vi "Write Outputs.vi"(8 "error in (no error)":errorcluster, 10 "Analog Outputs":sgl[](array[numeric]), 11 "An Out in":refnum<class "M5StackDAC2.lvclass">) -> (0 "error out":errorcluster, 3 "An Out out":refnum<class "M5StackDAC2.lvclass">)   [LabVIEW 2020, in "CTI-Peripheral.lvlib" / "M5StackDAC2.lvclass"]
uses:
  M5StackDAC2.lvclass
  M5StackDAC2.lvclass/M5StackDAC2.ctl
  CTI/I2C Connection/I2C Connection.lvclass/I2C Connection.ctl
  CTI/Session/I2C Write Data.vi
  CTI/I2C Connection/I2C Connection.lvclass
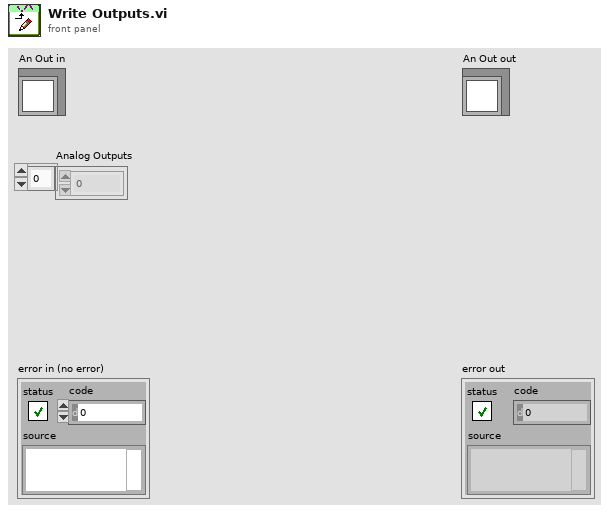
[diagram p1: front panel]
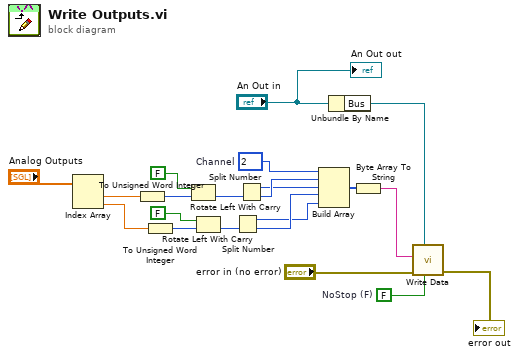
[diagram p0: block diagram]
diagram:
  w19 = u8 2  # Channel
  w20 = FALSE  # NoStop (F)
  n1 = Index Array(array="Analog Outputs") -> (element #1=w8:sgl, element #2=w7:sgl)  [unwired: 2 in]
  n2 = To Unsigned Word Integer(number=w8) -> (unsigned 16bit integer=w6:u16)
  n3 = To Unsigned Word Integer(number=w7) -> (unsigned 16bit integer=w5:u16)
  n4 = Rotate Left With Carry(2:w6, 3:FALSE ("carry")) -> (0:w17:u16)  [unwired: 1 out]
  n5 = Rotate Left With Carry(2:w5, 3:FALSE ("carry")) -> (0:w15:u16)  [unwired: 1 out]
  n6 = Split Number(x=w15) -> (hi(x)=w11:u8, lo(x)=w12:u8)
  n7 = Split Number(x=w17) -> (hi(x)=w13:u8, lo(x)=w14:u8)
  n8 = Build Array(w19, w14, w13, w12, w11) -> (w10:u8[])
  n9 = Unbundle By Name("An Out in") -> ("Bus"=w21:refnum<class "I2C Connection.lvclass">)
  n10 = Byte Array To String(unsigned byte array=w10) -> (string=w9:string)
  n11 = call "Write Data.vi"("NoStop (F)"=w20, "I2C Connection"=w21, "error in (no error)"="error in (no error)", "Data"=w9) -> ("error out"=→"error out":errorcluster)  [unwired: 7 in]
  "An Out out" <- "An Out in"
